vi "Check Current TurnTable Angle In Offset.vi"(8 "error in (no error)":errorcluster, 9 "Target Offset":dbl min=0.0, 10 "Current Angle":dbl, 11 "CO3000 in":refnum<class "CO3000.lvclass">) -> (0 "error out":errorcluster, 2 "In Offset Range?":bool, 3 "CO3000 out":refnum<class "CO3000.lvclass">)   [LabVIEW 2023, in "Turn Table and Mast.lvlib" / "CO3000.lvclass"]
uses:
  CO3000.lvclass
  CO3000.lvclass/CO3000.ctl
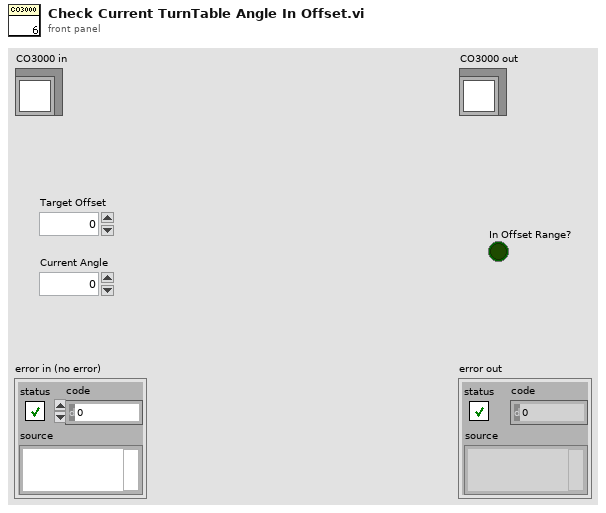
[diagram p1: front panel]
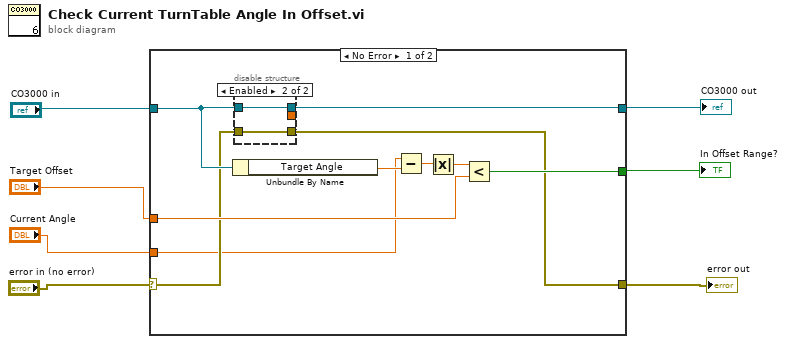
[diagram p0: block diagram]
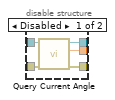
[diagram p2: hidden frame]
diagram:
  n1 = case shown="No Error" "error in (no error)" {
    selector: "error in (no error)" -> [w10 w26]
    tunnel: [w9 w26] -> w3
    tunnel: [w12 w25] -> w4
    tunnel: "CO3000 in" -> [w16 w25]
    tunnel: "Target Offset" -> [w13 _]
    tunnel: [w11 _] -> w5
    tunnel: "Current Angle" -> [w8 _]
    frame No Error {
      n2 = Unbundle By Name(w16) -> ("Target Angle"=w15:dbl)
      n3 = disable-structure shown="Enabled" {
        disable-tunnel: w16 -> [w22 w24]
        disable-tunnel: [w21 _] -> _
        disable-tunnel: [w20 w24] -> w12
        disable-tunnel: w10 -> [w19 w23]
        disable-tunnel: [w18 w23] -> w9
        frame Disabled {
          n4 = call-dynamic "Query Current Angle.vi"("error in (no error)"=w19, "CO3000 in"=w22) -> ("error out"=w18:errorcluster, "Current Angle"=w21:dbl, "CO3000 out"=w20:refnum<class "CO3000.lvclass">)  [unwired: 7 in]
        }
        frame Enabled {
        }
      }
      n5 = Subtract(x=w8, y=w15) -> (x-y=w17:dbl)
      n6 = Absolute Value(x=w17) -> (abs(x)=w14:dbl)
      n7 = Less?(x=w14, y=w13) -> (x < y?=w11:bool)
    }
    frame Error {
    }
  }
  "error out" <- w3
  "CO3000 out" <- w4
  "In Offset Range?" <- w5
